vi "Create subVI and deserialize.vi"(0 "VI in":refnum<vi>, 5 "Cluster Term Refnum":refnum<vi>, 7 "Name Out":string, 11 "error in (no error)":errorcluster) -> (15 "error out":errorcluster)   [LabVIEW 2021, in "Migrator.lvlib"]
uses:
  Migrator.lvlib
  <vilib>/Utility/miscctls.llb/LVPointTypeDef.ctl
  Path Functions/Path Functions.lvlib
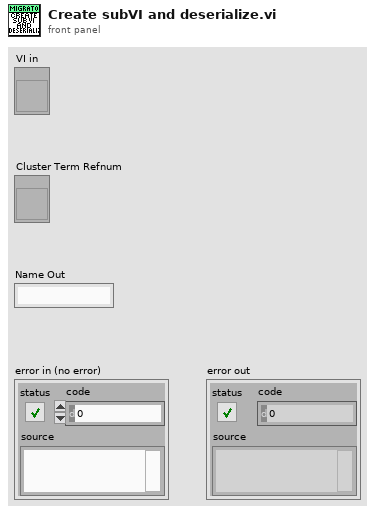
[diagram p1: front panel]
types:
  T1 = typedef "LVPointTypeDef.ctl" = cluster{"Horizontal":i16, "Vertical":i16}
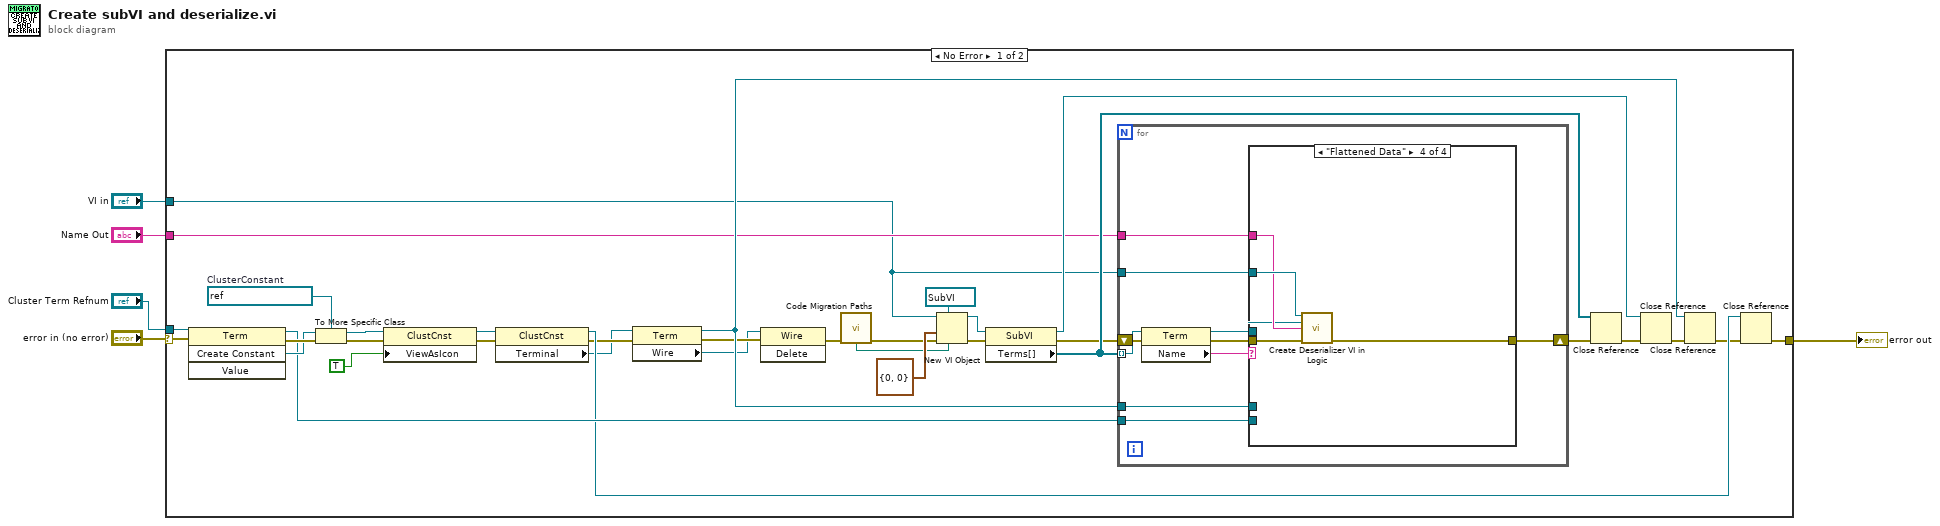
[diagram p0: block diagram]
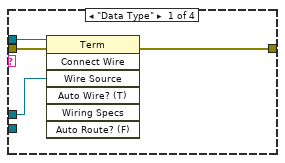
[diagram p2: hidden frame]
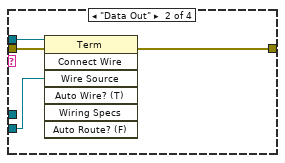
[diagram p3: hidden frame]
diagram:
  n1 = case shown="No Error" "error in (no error)" {
    selector: "error in (no error)" -> [w7 w64]
    tunnel: [w29 w64] -> w5
    tunnel: "Name Out" -> [w21 _]
    tunnel: "VI in" -> [w20 _]
    tunnel: "Cluster Term Refnum" -> [w6 _]
    frame No Error {
      w34 = refnum<vi> refnum  # ClusterConstant
      n2 = invoke class="Term" method="Create Constant"(reference=w6, error in=w7) -> (reference out=w30:refnum<vi>, error out=w36:errorcluster, "Create Constant"=w32:refnum<vi>)  [unwired: 2 in, 1 out]
      n3 = To More Specific Class(target class=w34, reference=w32, error in=w36) -> (specific class reference=w33:refnum<vi>, error out=w37:errorcluster)
      n4 = property class="ClustCnst"(reference=w33, error in=w37, "ViewAsIcon"=TRUE ("View As Icon")) -> (reference out=w38:refnum<vi>, error out=w39:errorcluster)
      n5 = property class="ClustCnst"(reference=w38, error in=w39) -> (reference out=w28:refnum<vi>, error out=w18:errorcluster, "Terminal"=w16:refnum<vi>)
      n6 = property class="Term"(reference=w16, error in=w18) -> (reference out=w31:refnum<vi>, error out=w19:errorcluster, "Wire"=w17:refnum<vi>)
      n7 = invoke class="Wire" method="Delete"(reference=w17, error in=w19) -> (error out=w8:errorcluster)  [unwired: 1 in, 2 out]
      n8 = call "Code Migration Paths.vi"("error in (no error)"=w8) -> ("Deserializer"=w9:path, "error out"=w10:errorcluster)  [unwired: 7 in, 6 out]
      n9 = New VI Object(vi object class=refnum<vi> refnum ("Other Refnum"), owner refnum=w20, position/next to=T1 {"Horizontal"=0, "Vertical"=0} ("location"), 6:w9, 8:w10) -> (object refnum=w13:refnum<vi>, 0:w14:errorcluster)  [unwired: 3 in]
      n10 = property class="SubVI"(reference=w13, error in=w14) -> (reference out=w25:refnum<vi>, error out=w15:errorcluster, "Terms[]"=w23:refnum<vi>[])
      n11 = for {
        tunnel: w23 -> [w46] mode=indexing
        shift-right: [w44] -> w22
        shift-left: w15 -> [w49]
        tunnel: w20 -> [w43]
        tunnel: w21 -> [w42]
        tunnel: w30 -> [w41]
        tunnel: w31 -> [w40]
        n12 = property class="Term"(reference=w46, error in=w49) -> (reference out=w45:refnum<vi>, error out=w48:errorcluster, "Name"=w47:string)
        n13 = case shown="\"Flattened Data\"" w47 {
          tunnel: w48 -> [w52 w57 w58 w63]
          tunnel: w45 -> [w53 w56 _ w60]
          tunnel: [w51 w55 w58 w59] -> w44
          tunnel: w43 -> [_ _ _ w62]
          tunnel: w42 -> [_ _ _ w61]
          tunnel: w41 -> [_ w54 _ _]
          tunnel: w40 -> [w50 _ _ _]
          frame "Data Type" {
            n14 = invoke class="Term" method="Connect Wire"(reference=w53, error in=w52, "Wire Source"=w50) -> (error out=w51:errorcluster)  [unwired: 4 in, 6 out]
          }
          frame "Data Out" {
            n15 = invoke class="Term" method="Connect Wire"(reference=w56, error in=w57, "Wire Source"=w54) -> (error out=w55:errorcluster)  [unwired: 4 in, 6 out]
          }
          frame Default {
          }
          frame "Flattened Data" {
            n16 = call "Create Deserializer VI in Logic.vi"("VI in"=w62, "Term Refnum"=w60, "Name Out"=w61, "error in (no error)"=w63) -> ("error out"=w59:errorcluster)  [unwired: 11 in]
          }
        }
      }
      n17 = Close Reference(reference=w23, error in (no error)=w22) -> (error out=w24:errorcluster)
      n18 = Close Reference(reference=w25, error in (no error)=w24) -> (error out=w26:errorcluster)
      n19 = Close Reference(reference=w31, error in (no error)=w26) -> (error out=w27:errorcluster)
      n20 = Close Reference(reference=w28, error in (no error)=w27) -> (error out=w29:errorcluster)
    }
    frame Error {
    }
  }
  "error out" <- w5
